vi "getConnectionPoint.vi"(0 "reference":refnum<class "ImplicitParameterNode.lvclass">, 1 "direction":refnum<class "Direction.lvclass">, 5 "error in (no error)":errorcluster) -> (14 "reference out":refnum<class "ImplicitParameterNode.lvclass">, 15 "point2D":T1 {"y" format="%.2f"; "x" format="%.2f"}, 19 "error out":errorcluster)   [LabVIEW 2020, in "ImplicitParameterNode.lvclass"]
doc: "public Point2D getConnectionPoint(Direction d)"
uses:
  <resource>/Framework/Providers/Open_GDS/UML/ImplicitParameterNode_class/ImplicitParameterNode.lvclass
  C:/Program Files (x86)/National Instruments/LabVIEW 2020/resource/Framework/Providers/Open_GDS/UML/RectangularNode_class/RectangularNode.lvclass
  <resource>/Framework/Providers/Open_GDS/UML/Direction_class/Direction.lvclass
  <resource>/Framework/Providers/Open_GDS/UML/General/Point/Point Point2D.ctl
  <resource>/Framework/Providers/Open_GDS/UML/RectangularNode_class/RectangularNode.lvclass
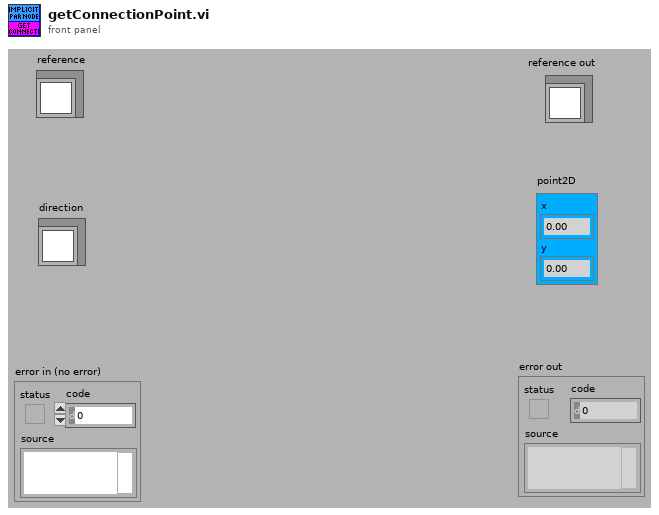
[diagram p1: front panel]
types:
  T1 = typedef "Point Point2D.ctl" = cluster{"x":dbl, "y":dbl}
  T2 = typedef "ImplicitParameterNode.lvclass/ObjectAttributes.ctl" = cluster{"topHeight":dbl, "name":refnum<class "MultiLineString.lvclass">, "DEFAULT_TOP_HEIGHT":i32, "DEFAULT_WIDTH":i32, "DEFAULT_HEIGHT":i32}
  T3 = typedef "RectangularNode.lvclass/ObjectAttributes.ctl" = cluster{"bounds":T4}
  T4 = typedef "Rectangle Rectangle2D.ctl" = cluster{"x":dbl, "y":dbl, "width":dbl, "height":dbl}
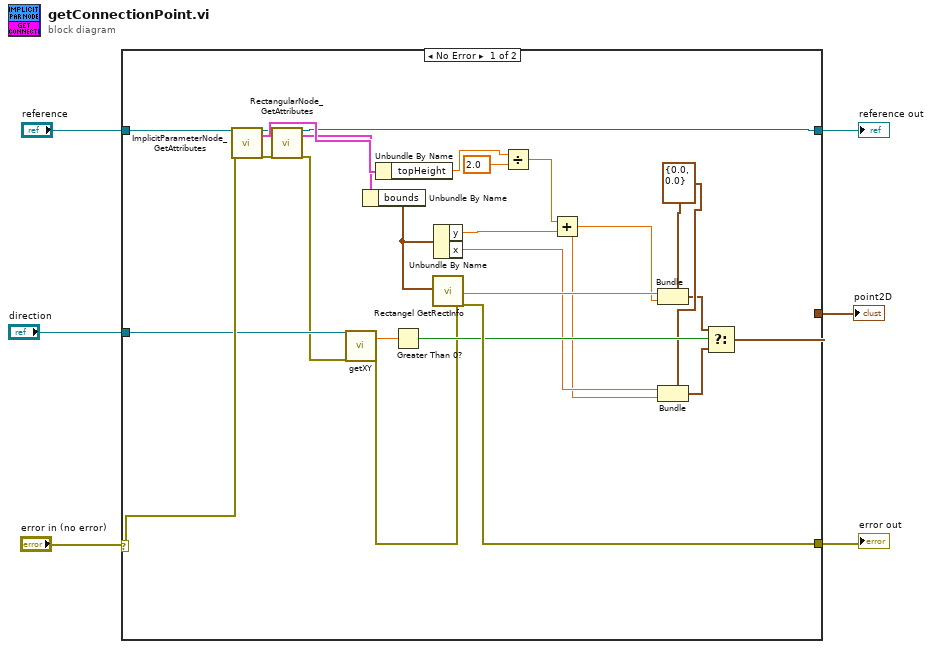
[diagram p0: block diagram]
diagram:
  n1 = case shown="No Error" "error in (no error)" {
    selector: "error in (no error)" -> [w29 w32]
    tunnel: "reference" -> [w31 w33]
    tunnel: [w30 w32] -> w5
    tunnel: [w8 w33] -> w4
    tunnel: [w28 _] -> w2
    tunnel: "direction" -> [w27 _]
    frame No Error {
      w24 = T1 {"x"=0.0, "y"=0.0} ("point2D")
      n2 = call <resource>:"ImplicitParameterNode_GetAttributes.vi"("reference in"=w31, "error in (no error)"=w29) -> ("reference out"=w11:refnum<class "ImplicitParameterNode.lvclass">, "Data"=w12:T2, "error out"=w10:errorcluster)  [unwired: 1 in, 14 out]
      n3 = call <resource>:"RectangularNode_GetAttributes.vi"("reference in"=w11, "error in (no error)"=w10) -> ("reference out"=w8:refnum<class "ImplicitParameterNode.lvclass">, "Data"=w7:T3, "error out"=w9:errorcluster)  [unwired: 14 in, 1 out]
      n4 = call <resource>:"getXY.vi"("reference"=w27, "error in (no error)"=w9) -> ("x"=w26:dbl, "error out"=w13:errorcluster)  [unwired: 16 out]
      n5 = Unbundle By Name(w7) -> ("bounds"=w21:T4)
      n6 = Unbundle By Name(w12) -> ("topHeight"=w19:dbl)
      n7 = Greater Than 0?(x=w26) -> (x > 0?=w25:bool)
      n8 = call <resource>:"Rectangel GetRectInfo.vi"("bounds"=w21, "error in (no error)"=w13) -> ("maxX"=w22:dbl, "error out"=w30:errorcluster)  [unwired: 16 out]
      n9 = Unbundle By Name(w21) -> ("y"=w20:dbl, "x"=w15:dbl)
      n10 = Divide(x=w19, y=2.0) -> (x/y=w17:dbl)
      n11 = Add(x=w17, y=w20) -> (x+y=w14:dbl)
      n12 = Bundle(cluster=w24, "x"=w22, "y"=w14) -> (w23:T1)
      n13 = Bundle(cluster=w24, "x"=w15, "y"=w14) -> (w16:T1)
      n14 = Select(t=w23, s=w25, f=w16) -> (s? t:f=w28:T1)
    }
    frame Error {
    }
  }
  "reference out" <- w4
  "error out" <- w5
  "point2D" <- w2
